vi "FSK Modulator.vi"(0 "Baseband Signal":dbl[](array[numeric]), 1 "Sampling Frequency(Fs)":dbl, 2 "Lower Frequency (f0)":dbl, 3 "Higher Frequency(f1)":dbl, 4 "Carrier Amplitude(A)":dbl) -> (5 "FSK Modulated Signal":dbl[](array[numeric]))   [LabVIEW 2026]
panel:
  out "FSK Modulated Waveform":dbl[](graph)
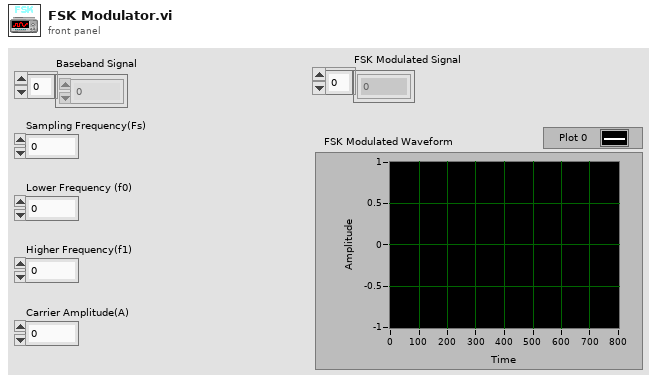
[diagram p1: front panel]
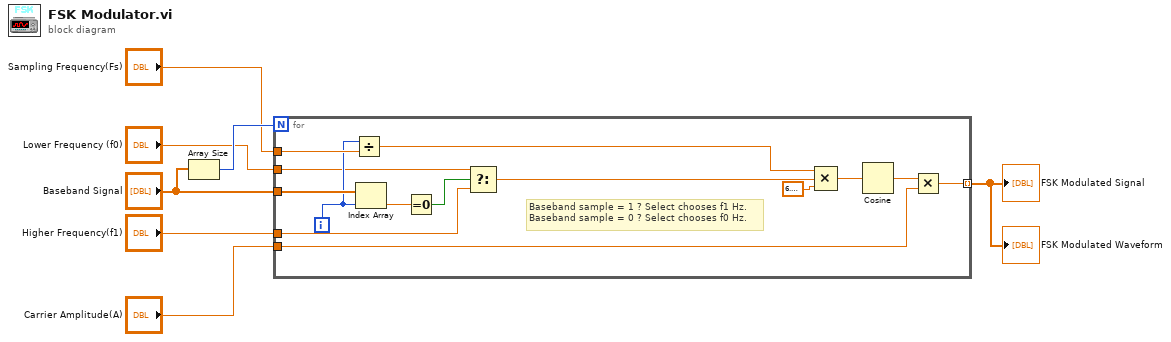
[diagram p0: block diagram]
diagram:
  n1 = Array Size(array="Baseband Signal") -> (size(s)=w7:i32)
  n2 = for {
    N: w7 -> [_]
    tunnel: "Sampling Frequency(Fs)" -> [w21]
    tunnel: "Baseband Signal" -> [w19]
    tunnel: "Lower Frequency (f0)" -> [w15]
    tunnel: "Higher Frequency(f1)" -> [w14]
    tunnel: [w10] -> w2 mode=indexing
    tunnel: "Carrier Amplitude(A)" -> [w8]
    i -> [w18]
    # "Baseband sample = 1 ? Select chooses f1 Hz.\nBaseband sample = 0 ? Select chooses f0 Hz."
    n3 = Divide(x=w18, y=w21) -> (x/y=w20:dbl)
    n4 = Index Array(array=w19, index=w18) -> (element=w17:dbl)
    n5 = Equal To 0?(x=w17) -> (x = 0?=w16:bool)
    n6 = Select(t=w15, s=w16, f=w14) -> (s? t:f=w13:dbl)
    n7 = Compound Arithmetic op=MULTIPLY(w20, w13, 6.283185307179586) -> (w11:dbl)
    n8 = Cosine(x=w11) -> (cos(x)=w9:dbl)
    n9 = Multiply(x=w9, y=w8) -> (x*y=w10:dbl)
  }
  "FSK Modulated Signal" <- w2
  "FSK Modulated Waveform" <- w2
